vi "Map to List of Ctrl.vi"(10 "CTRLs":map{path, T1[]}(c390), 11 "FP.Tr":map{string, T2}(c390)) -> (3 "List of Ctrl":string[][](array[string]))   [LabVIEW 2019, in "Language Editor.lvlib"]
doc: "- - -\nCopyright (c) 2026, Merecs Engineering GmbH"
uses:
  Language Editor.lvlib
  type defs/Cluster Translations.ctl
  Language Selection/TypeDefs/Cluster PropertyTranslation.ctl
  Language Selection/TypeDefs/Enum Property Type.ctl
  type defs/Cluster VI controls.ctl
  Language Selection/Language Selection.lvlib
panel:
  # "Connector Pane"
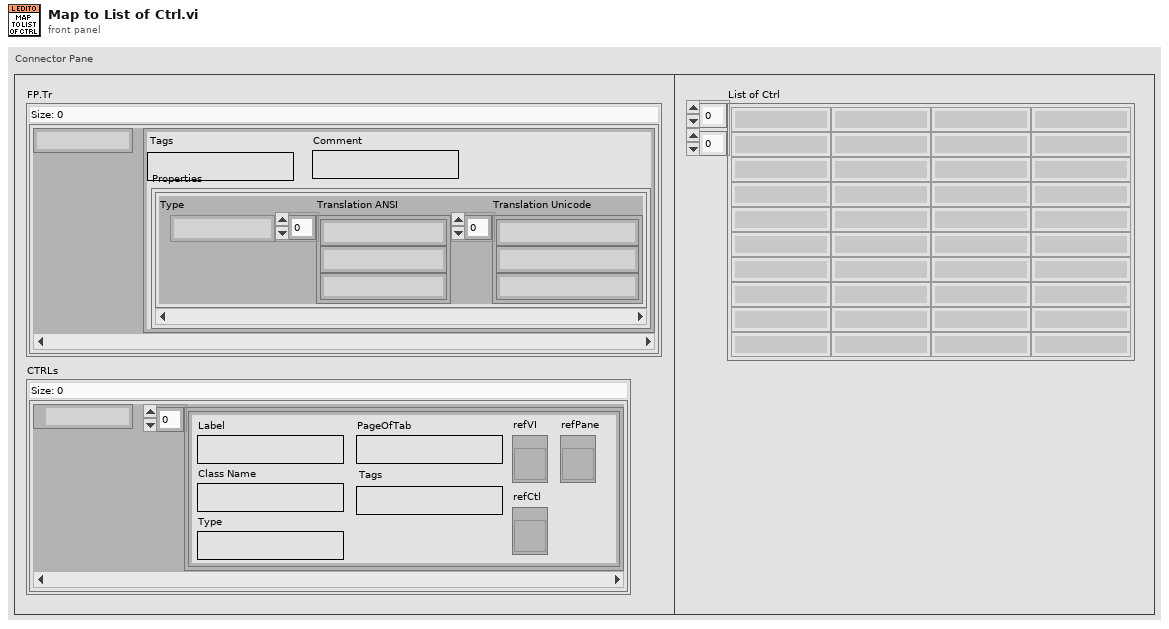
[diagram p1: front panel]
types:
  T1 = typedef "Language Editor.lvlib/Cluster VI controls.ctl" = cluster{"Label":string, "Class Name":string, "Type":string, "Tags":string, "refVI":refnum<vi>, "refCtl":refnum<vi>, "PageOfTab":string, "refPane":refnum<vi>}
  T2 = typedef "Language Editor.lvlib/Cluster Translations.ctl" = cluster{"Tags":string, "Comment":string, "Properties":T3[]}
  T3 = typedef "Language Selection.lvlib/Cluster PropertyTranslation.ctl" = cluster{"Type":T4, "Translation ANSI":string[], "Translation Unicode":string[]}
  T4 = typedef "Language Selection.lvlib/Enum Property Type.ctl" = enum16{"NA", "Caption", "String Value", "Boolean Text", "Ring Strings", "1D Array Elements", "2D Array Elements", "(MC)Listbox Header", "(MC)Listbox Items", "Tab Pages Names", "X & Y GraphChart", "Plot Names", "Table Headers", "Table Items", "TipStrip", "Combobox Strings", "Cursor Name", "Tree Col Headers"}
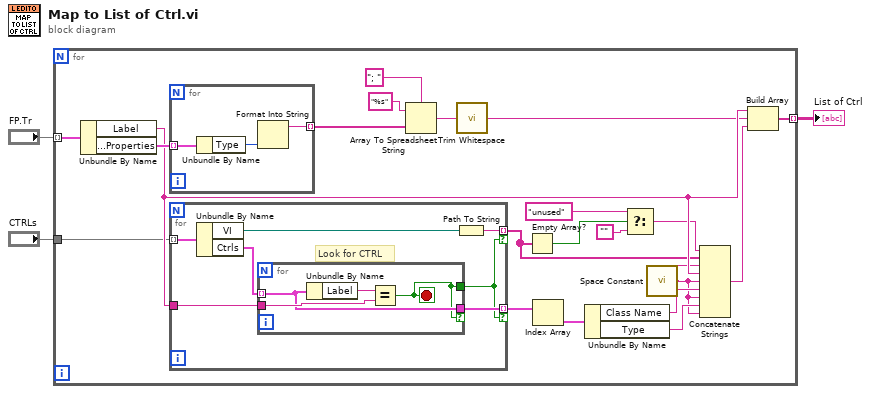
[diagram p0: block diagram]
diagram:
  n1 = for {
    tunnel: "FP.Tr" -> [w24] mode=indexing
    tunnel: [w23] -> w3 mode=indexing
    tunnel: "CTRLs" -> [w15]
    n2 = Unbundle By Name(w24) -> ("Label"=w21:string, "Translation.Properties"=w22:T3[])
    n3 = for {
      tunnel: w22 -> [w38] mode=indexing
      tunnel: [w36] -> w20 mode=indexing
      n4 = Unbundle By Name(w38) -> ("Type"=w37:T4)
      n5 = Format Into String(w37) -> (resulting string=w36:string)  [unwired: 3 in, 1 out]
    }
    n6 = for {
      tunnel: w15 -> [w31] mode=indexing
      tunnel: w21 -> [w30]
      tunnel: [w27] -> w14 mode=indexing if=w25
      tunnel: [w26] -> w10 mode=indexing if=w25
      # "Look for CTRL"
      n7 = Unbundle By Name(w31) -> ("VI"=w29:path, "Ctrls"=w28:T1[])
      n8 = for {
        tunnel: w28 -> [w33] mode=indexing
        tunnel: w30 -> [w35]
        tunnel: [w32] -> w25
        tunnel: [w33] -> w27 if=w32
        stop <- w32 stop-if-true
        n9 = Unbundle By Name(w33) -> ("Label"=w34:string)
        n10 = Equal?(x=w34, y=w35) -> (x = y?=w32:bool)
      }
      n11 = Path To String(path=w29) -> (string=w26:string)
    }
    n12 = Array To Spreadsheet String(delimiter (Tab)="; ", array=w20, 3:"%s" ("format string")) -> (spreadsheet string=w19:string)
    n13 = call <vilib>:"Trim Whitespace.vi"("string"=w19) -> ("trimmed string"=w17:string)  [unwired: 1 in]
    n14 = Empty Array?(array=w10) -> (empty?=w8:bool)
    n15 = Index Array(array=w14) -> (element=w13:T1)  [unwired: 1 in]
    n16 = Unbundle By Name(w13) -> ("Class Name"=w12:string, "Type"=w11:string)
    n17 = Select(t="unused", s=w8, f="") -> (s? t:f=w9:string)
    n18 = call <vilib>:"Space Constant.vi"() -> ("String"=w5:string)
    n19 = Concatenate Strings(w9, w10, w5, w21, w5, w12, w5, w11, w5) -> (w4:string)
    n20 = Build Array(w21, w17, w4) -> (w23:string[])
  }
  "List of Ctrl" <- w3
